vi "ACK.vi"(6 "timeout (ms) [100]":i32=100, 8 "error in (no error)":errorcluster, 11 "Instrument in":refnum<class "Instrument.lvclass">) -> (0 "error out":errorcluster, 2 "ACK":string, 3 "Instrument out":refnum<class "Instrument.lvclass">)   [LabVIEW 2019, in "Instrument.lvlib" / "Instrument.lvclass"]
doc: "Send \"ACK\" command to remote Instrument to test connectivity."
uses:
  Instrument.lvclass
  Typedefs/Instrument.Commands--Enum.ctl
  f7bd5210-6898-44d9-a8a8-036b7bc7be21.vi
  f7bd5210-6898-44d9-a8a8-036b7bc7be21.vi/ed14601c-1b73-4eb4-becb-0f2adfab3405.vi
  f7bd5210-6898-44d9-a8a8-036b7bc7be21.vi/a7fe8284-0d85-4ee4-ad7b-3e8a282efae9.vi
  <vilib>/Utility/Data Type/Get Type Information.vi
  <vilib>/JDP Science/JSONtext/JSON text to Variant.vi
  <vilib>/JDP Science/JSONtext/LVClass Serializer/JSONtext LVClass Serializer.lvclass
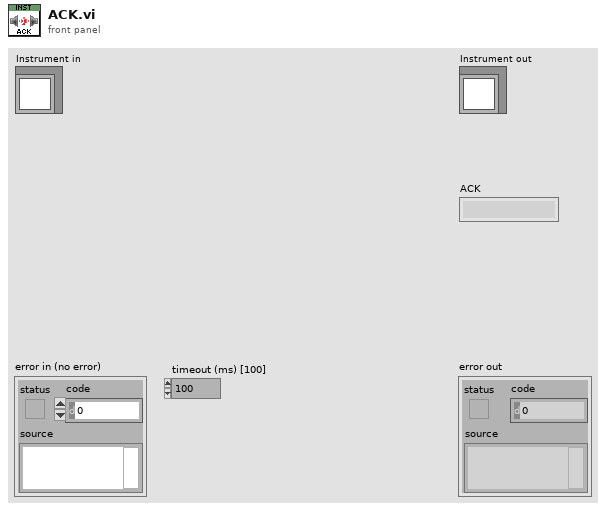
[diagram p1: front panel]
types:
  T1 = typedef "Instrument.lvlib/Instrument.lvclass/Instrument.Commands--Enum.ctl" = enum16{"ACK", "HELP", "IDN", "getAll", "getAllData"}
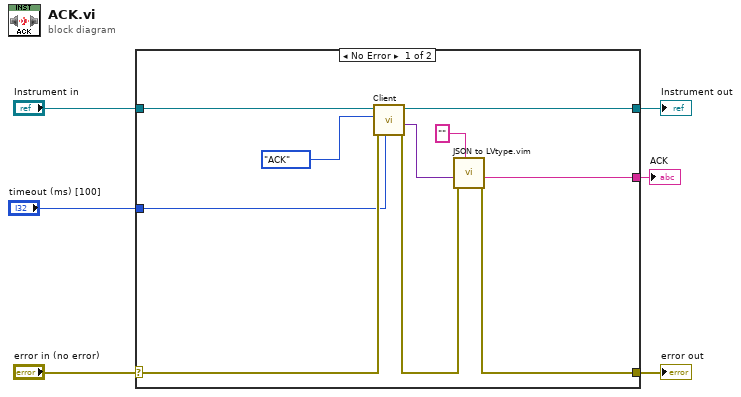
[diagram p0: block diagram]
diagram:
  n1 = case shown="No Error" "error in (no error)" {
    selector: "error in (no error)" -> [w14 w18]
    tunnel: [w10 w18] -> w5
    tunnel: [w16 w17] -> w3
    tunnel: "Instrument in" -> [w15 w17]
    tunnel: [w9 _] -> w2
    tunnel: "timeout (ms) [100]" -> [w7 _]
    frame No Error {
      n2 = call-dynamic "Client.vi"("timeout (ms) [500]"=w7, "error in (no error)"=w14, "Command in"=Instrument.Commands--Enum."ACK" ("Commands"), "Instrument in"=w15) -> ("error out"=w8:errorcluster, "Data out"=w11:variant, "Instrument out"=w16:refnum<class "Instrument.lvclass">)  [unwired: 4 in, 1 out]
      n3 = call "JSON to LVtype.vim"("type"="" ("Commands"), "error in (no error)"=w8, "JSON Data in"=w11) -> ("error out"=w10:errorcluster, "Data out"=w9:string)  [unwired: 7 in]
    }
    frame Error {
    }
  }
  "error out" <- w5
  "Instrument out" <- w3
  "ACK" <- w2
